vi "Run All.vi"(8 "Error In":errorcluster) -> (0 "Error Out":errorcluster)   [LabVIEW 2018, in "Tests.lvlib"]
uses:
  Tests.lvlib
  Support/Secret Types.ctl
  SSH/SSH.lvlib
  Session/Session.lvlib
  <vilib>/addons/_JKI Toolkits/Caraya/classes/Test/Test.lvclass
  Known Hosts/Known Hosts.lvlib
  Known Host/Known Host.lvlib
  SFTP File/SFTP File.lvlib
  SFTP Attributes/SFTP Attributes.lvlib
  SFTP/SFTP.lvlib
  SFTP Directory/SFTP Directory.lvlib
  File Info/File Info.lvlib
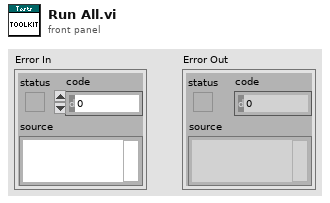
[diagram p1: front panel]
types:
  T1 = typedef "Tests.lvlib/Secret Types.ctl" = enum16{"Passphrase", "Password"}
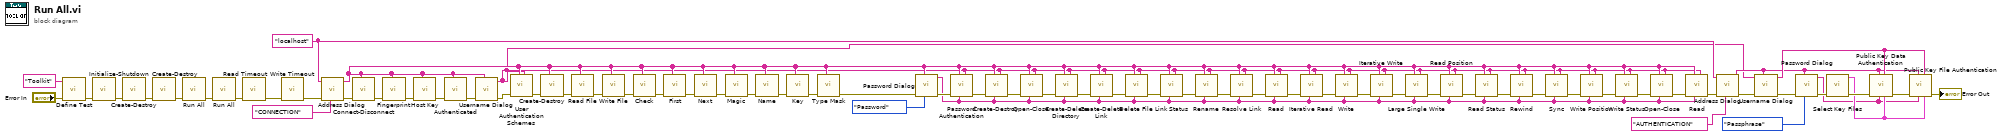
[diagram p0: block diagram]
diagram:
  w53 = "localhost" ("Address")
  n1 = call <vilib>:"Define Test.vi"("error in (no error)"="Error In", "Label (VI Title)"="Toolkit") -> ("error out"=w67:errorcluster)  [unwired: 9 in]
  n2 = call "Initialize-Shutdown.vi"("Error In"=w67) -> ("Error Out"=w68:errorcluster)  [unwired: 10 in]
  n3 = call "Create-Destroy.vi"("Error In"=w68) -> ("Error Out"=w41:errorcluster)  [unwired: 10 in]
  n4 = call "Create-Destroy.vi"("Error In"=w41) -> ("Error Out"=w30:errorcluster)  [unwired: 10 in]
  n5 = call "Run All.vi"("Error In"=w30) -> ("Error Out"=w12:errorcluster)  [unwired: 10 in]
  n6 = call "Run All.vi"("Error In"=w12) -> ("Error Out"=w3:errorcluster)  [unwired: 10 in]
  n7 = call "Read Timeout.vi"("Error In"=w3) -> ("Error Out"=w2:errorcluster)  [unwired: 10 in]
  n8 = call "Write Timeout.vi"("Error In"=w2) -> ("Error Out"=w1:errorcluster)  [unwired: 10 in]
  n9 = call "Address Dialog.vi"("Title"="CONNECTION", "Error In"=w1, "Address In"=w53) -> ("Error Out"=w54:errorcluster, "Address Out"=w5:string)  [unwired: 7 in]
  n10 = call "Connect-Disconnect.vi"("Address"=w5, "Error In"=w54) -> ("Error Out"=w38:errorcluster)  [unwired: 9 in]
  n11 = call "Fingerprint.vi"("Address"=w5, "Error In"=w38) -> ("Error Out"=w45:errorcluster)  [unwired: 9 in]
  n12 = call "Host Key.vi"("Address"=w5, "Error In"=w45) -> ("Error Out"=w44:errorcluster)  [unwired: 9 in]
  n13 = call "Authenticated.vi"("Address"=w5, "Error In"=w44) -> ("Error Out"=w62:errorcluster)  [unwired: 9 in]
  n14 = call "Username Dialog.vi"("Address"=w5, "Error In"=w62) -> ("Error Out"=w61:errorcluster, "Username Out"=w4:string)  [unwired: 8 in]
  n15 = call "User Authentication Schemes.vi"("Username"=w4, "Address"=w5, "Error In"=w61) -> ("Error Out"=w48:errorcluster)  [unwired: 8 in]
  n16 = call "Create-Destroy.vi"("Address"=w5, "Error In"=w48) -> ("Error Out"=w46:errorcluster)  [unwired: 9 in]
  n17 = call "Read File.vi"("Address"=w5, "Error In"=w46) -> ("Error Out"=w43:errorcluster)  [unwired: 9 in]
  n18 = call "Write File.vi"("Address"=w5, "Error In"=w43) -> ("Error Out"=w42:errorcluster)  [unwired: 9 in]
  n19 = call "Check.vi"("Address"=w5, "Error In"=w42) -> ("Error Out"=w37:errorcluster)  [unwired: 9 in]
  n20 = call "First.vi"("Address"=w5, "Error In"=w37) -> ("Error Out"=w36:errorcluster)  [unwired: 9 in]
  n21 = call "Next.vi"("Address"=w5, "Error In"=w36) -> ("Error Out"=w35:errorcluster)  [unwired: 9 in]
  n22 = call "Magic.vi"("Address"=w5, "Error In"=w35) -> ("Error Out"=w34:errorcluster)  [unwired: 9 in]
  n23 = call "Name.vi"("Address"=w5, "Error In"=w34) -> ("Error Out"=w33:errorcluster)  [unwired: 9 in]
  n24 = call "Key.vi"("Address"=w5, "Error In"=w33) -> ("Error Out"=w32:errorcluster)  [unwired: 9 in]
  n25 = call "Type Mask.vi"("Address"=w5, "Error In"=w32) -> ("Error Out"=w31:errorcluster)  [unwired: 9 in]
  n26 = call "Password Dialog.vi"("Secret Type"=Secret_Types."Password", "Address"=w5, "Error In"=w31) -> ("Error Out"=w40:errorcluster, "Password Out"=w6:string)  [unwired: 7 in]
  n27 = call "Password Authentication.vi"("Username"=w4, "Password"=w6, "Address"=w5, "Error In"=w40) -> ("Error Out"=w29:errorcluster)  [unwired: 7 in]
  n28 = call "Create-Destroy.vi"("Username"=w4, "Password"=w6, "Address"=w5, "Error In"=w29) -> ("Error Out"=w28:errorcluster)  [unwired: 7 in]
  n29 = call "Open-Close.vi"("Username"=w4, "Password"=w6, "Address"=w5, "Error In"=w28) -> ("Error Out"=w27:errorcluster)  [unwired: 7 in]
  n30 = call "Create-Delete Directory.vi"("Username"=w4, "Password"=w6, "Address"=w5, "Error In"=w27) -> ("Error Out"=w26:errorcluster)  [unwired: 7 in]
  n31 = call "Create-Delete Link.vi"("Username"=w4, "Password"=w6, "Address"=w5, "Error In"=w26) -> ("Error Out"=w25:errorcluster)  [unwired: 7 in]
  n32 = call "Delete File.vi"("Username"=w4, "Password"=w6, "Address"=w5, "Error In"=w25) -> ("Error Out"=w24:errorcluster)  [unwired: 7 in]
  n33 = call "Link Status.vi"("Username"=w4, "Password"=w6, "Address"=w5, "Error In"=w24) -> ("Error Out"=w23:errorcluster)  [unwired: 7 in]
  n34 = call "Rename.vi"("Username"=w4, "Password"=w6, "Address"=w5, "Error In"=w23) -> ("Error Out"=w22:errorcluster)  [unwired: 7 in]
  n35 = call "Resolve Link.vi"("Username"=w4, "Password"=w6, "Address"=w5, "Error In"=w22) -> ("Error Out"=w21:errorcluster)  [unwired: 7 in]
  n36 = call "Read.vi"("Username"=w4, "Password"=w6, "Address"=w5, "Error In"=w21) -> ("Error Out"=w11:errorcluster)  [unwired: 7 in]
  n37 = call "Iterative Read.vi"("Username"=w4, "Password"=w6, "Address"=w5, "Error In"=w11) -> ("Error Out"=w10:errorcluster)  [unwired: 7 in]
  n38 = call "Write.vi"("Username"=w4, "Password"=w6, "Address"=w5, "Error In"=w10) -> ("Error Out"=w9:errorcluster)  [unwired: 7 in]
  n39 = call "Iterative Write.vi"("Username"=w4, "Password"=w6, "Address"=w5, "Error In"=w9) -> ("Error Out"=w8:errorcluster)  [unwired: 7 in]
  n40 = call "Large Single Write.vi"("Username"=w4, "Password"=w6, "Address"=w5, "Error In"=w8) -> ("Error Out"=w7:errorcluster)  [unwired: 7 in]
  n41 = call "Read Position.vi"("Username"=w4, "Password"=w6, "Address"=w5, "Error In"=w7) -> ("Error Out"=w20:errorcluster)  [unwired: 7 in]
  n42 = call "Read Status.vi"("Username"=w4, "Password"=w6, "Address"=w5, "Error In"=w20) -> ("Error Out"=w19:errorcluster)  [unwired: 7 in]
  n43 = call "Rewind.vi"("Username"=w4, "Password"=w6, "Address"=w5, "Error In"=w19) -> ("Error Out"=w18:errorcluster)  [unwired: 7 in]
  n44 = call "Sync.vi"("Username"=w4, "Password"=w6, "Address"=w5, "Error In"=w18) -> ("Error Out"=w17:errorcluster)  [unwired: 7 in]
  n45 = call "Write Position.vi"("Username"=w4, "Password"=w6, "Address"=w5, "Error In"=w17) -> ("Error Out"=w16:errorcluster)  [unwired: 7 in]
  n46 = call "Write Status.vi"("Username"=w4, "Password"=w6, "Address"=w5, "Error In"=w16) -> ("Error Out"=w15:errorcluster)  [unwired: 7 in]
  n47 = call "Open-Close.vi"("Username"=w4, "Password"=w6, "Address"=w5, "Error In"=w15) -> ("Error Out"=w14:errorcluster)  [unwired: 7 in]
  n48 = call "Read.vi"("Username"=w4, "Password"=w6, "Address"=w5, "Error In"=w14) -> ("Error Out"=w13:errorcluster)  [unwired: 7 in]
  n49 = call "Address Dialog.vi"("Title"="AUTHENTICATION", "Error In"=w13, "Address In"=w53) -> ("Error Out"=w57:errorcluster, "Address Out"=w52:string)  [unwired: 7 in]
  n50 = call "Username Dialog.vi"("Address"=w52, "Error In"=w57, "Username In"=w4) -> ("Error Out"=w56:errorcluster, "Username Out"=w55:string)  [unwired: 7 in]
  n51 = call "Password Dialog.vi"("Secret Type"=Secret_Types."Passphrase", "Address"=w52, "Error In"=w56) -> ("Error Out"=w59:errorcluster, "Password Out"=w58:string)  [unwired: 7 in]
  n52 = call "Select Key Files.vi"("Error In"=w59) -> ("Error Out"=w63:errorcluster, "Key Files Out"=w60:cluster{"Private":path, "Public":path})  [unwired: 9 in]
  n53 = call "Public Key Data Authentication.vi"("Key Files"=w60, "Username"=w55, "Passphrase"=w58, "Address"=w52, "Error In"=w63) -> ("Error Out"=w64:errorcluster)  [unwired: 6 in]
  n54 = call "Public Key File Authentication.vi"("Key Files"=w60, "Username"=w55, "Passphrase"=w58, "Address"=w52, "Error In"=w64) -> ("Error Out"=→"Error Out":errorcluster)  [unwired: 6 in]
